vi "KeyToVirtualKey.vi"(11 "keyType Recorded":T1=enum."1") -> (2 "Unimplemented":bool, 3 "Virtual Key":T2=164)   [LabVIEW 2026]
uses:
  replay/KeyboardReplayKey.ctl
  UserEventRecorder/KeyType.ctl
panel:
  in  "\"":bool
  in  ",":bool
  in  ".":bool
  in  "/":bool
  in  "]":bool
  in  "\\":bool
  in  "-":bool
  in  "=":bool
  in  "[":bool
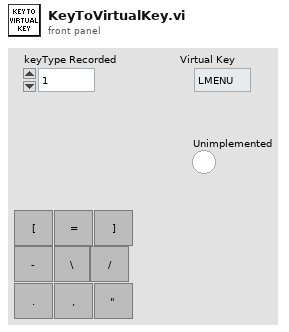
[diagram p1: front panel]
types:
  T1 = typedef "KeyType.ctl" = enum16{"0", "1", "2", "3", "4", "5", "6", "7", "8", "9", "A", "B", "C", "D", "E", "F", "G", "H", "I", "J", "K", "L", "M", "N", "O", "P", "Q", "R", "S", "T", "U", "V", "W", "X", "Y", "Z", "F1", "F2", "F3", "F4", "F5", "F6", "F7", "F8", "F9", "F10", "F11", "F12", "F13", "F14", "F15", "ADD", "BACK", "BACKSLASH", "CAPITAL", "COMMA", "DECIMAL", "DELETE", "DIVIDE", "DOWN", "END", "EQUALS", "ESCAPE", "GRAVE (`)", "HOME", "INSERT", "LBRACKET", "LCONTROL", "LEFT", "L ALT", "LSHIFT", "LWIN", "MINUS", "MULTIPLY", "NEXT", "NUMLOCK", "NUMPAD_0", "NUMPAD_1", "NUMPAD_2", "NUMPAD_3", "NUMPAD_4", "NUMPAD_5", "NUMPAD_6", "NUMPAD_7", "NUMPAD_8", "NUMPAD_9", "PAUSE", "PERIOD", "PRIOR (PG UP)", "RBRACKET", "RCONTROL", "RETURN", "RIGHT", "R ALT", "RSHIFT", "RWIN", "SCROLL", "SEMICOLON", "SLASH", "SPACE", "SUBTRACT", "TAB", "UP", "ENTER (num pad)", "' (quote)"}
  T2 = typedef "KeyboardReplayKey.ctl" = u8
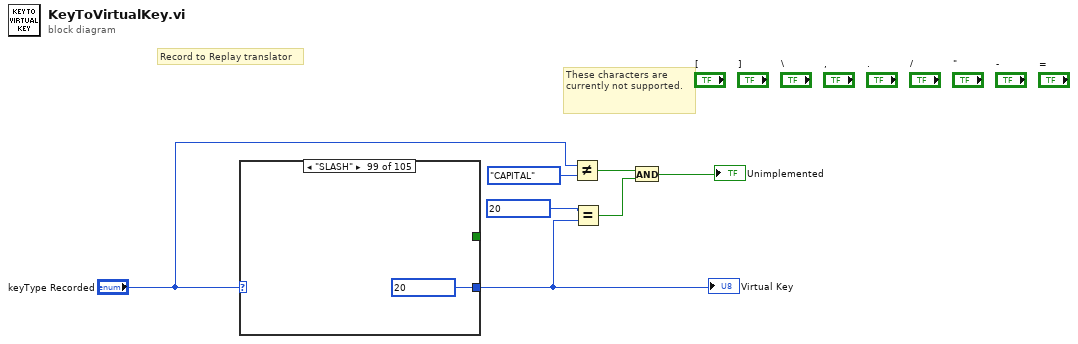
[diagram p0: block diagram]
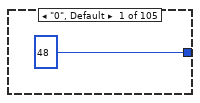
[diagram p2: hidden frame]
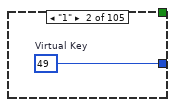
[diagram p3: hidden frame]
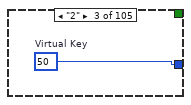
[diagram p4: hidden frame]
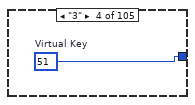
[diagram p5: hidden frame]
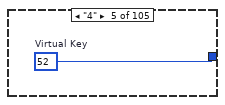
[diagram p6: hidden frame]
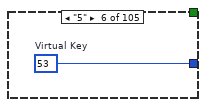
[diagram p7: hidden frame]
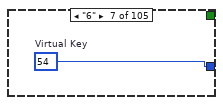
[diagram p8: hidden frame]
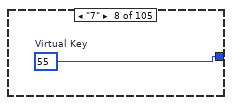
[diagram p9: hidden frame]
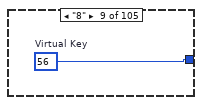
[diagram p10: hidden frame]
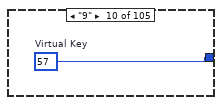
[diagram p11: hidden frame]
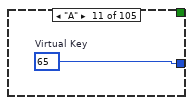
[diagram p12: hidden frame]
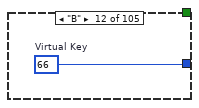
[diagram p13: hidden frame]
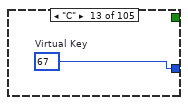
[diagram p14: hidden frame]
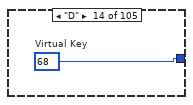
[diagram p15: hidden frame]
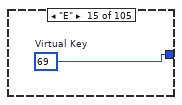
[diagram p16: hidden frame]
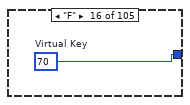
[diagram p17: hidden frame]
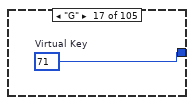
[diagram p18: hidden frame]
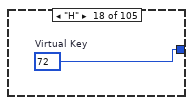
[diagram p19: hidden frame]
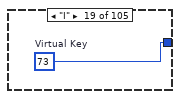
[diagram p20: hidden frame]
diagram:
  # "These characters are\ncurrently not supported."
  # "Record to Replay translator"
  n1 = case shown="\"SLASH\"" "keyType Recorded" {
    tunnel: [T2 48 ("Virtual Key") w9 w10 w11 w12 w13 w14 w15 w16 w17 w18 w19 w20 w21 w22 w23 w24 w25 w26 w27 w28 w29 w30 w31 w32 w33 w34 w35 w36 w37 w38 w39 w40 w41 w42 w43 w44 w45 w46 w47 w48 w49 w50 w51 w52 w53 w54 w55 w56 w57 w58 w59 w60 T2 20 ("Virtual Key") w63 T2 20 ("Virtual Key") w65 w66 w67 w68 w69 T2 20 ("Virtual Key") w71 T2 20 ("Virtual Key") w73 w74 T2 20 ("Virtual Key") w76 w77 w78 T2 160 ("Virtual Key") T2 91 ("Virtual Key") T2 109 ("Virtual Key") T2 106 ("Virtual Key") T2 34 ("Virtual Key") T2 144 ("Virtual Key") T2 96 ("Virtual Key") T2 97 ("Virtual Key") T2 98 ("Virtual Key") T2 99 ("Virtual Key") T2 100 ("Virtual Key") T2 101 ("Virtual Key") T2 102 ("Virtual Key") T2 103 ("Virtual Key") T2 104 ("Virtual Key") T2 105 ("Virtual Key") T2 19 ("Virtual Key") T2 20 ("Virtual Key") T2 33 ("Virtual Key") T2 20 ("Virtual Key") T2 163 ("Virtual Key") T2 43 ("Virtual Key") T2 39 ("Virtual Key") T2 165 ("Virtual Key") T2 161 ("Virtual Key") T2 92 ("Virtual Key") T2 145 ("Virtual Key") T2 164 ("Virtual Key") T2 20 ("Virtual Key") T2 32 ("Virtual Key") T2 109 ("Virtual Key") T2 9 ("Virtual Key") T2 38 ("Virtual Key") T2 20 ("Virtual Key") T2 20 ("Virtual Key")] -> w5
    tunnel: [_ _ _ _ _ _ _ _ _ _ _ _ _ _ _ _ _ _ _ _ _ _ _ _ _ _ _ _ _ _ _ _ _ _ _ _ _ _ _ _ _ _ _ _ _ _ _ _ _ _ _ _ _ w62 _ _ _ _ _ _ _ _ _ _ _ _ _ _ _ _ _ _ _ _ _ _ _ _ _ _ _ _ _ _ _ _ _ _ _ _ _ _ _ _ _ _ _ _ _ _ _ _ _ _ _] -> _
    frame "0", Default {
    }
    frame "1" {
      w9 = T2 49  # Virtual Key
    }
    frame "2" {
      w10 = T2 50  # Virtual Key
    }
    frame "3" {
      w11 = T2 51  # Virtual Key
    }
    frame "4" {
      w12 = T2 52  # Virtual Key
    }
    frame "5" {
      w13 = T2 53  # Virtual Key
    }
    frame "6" {
      w14 = T2 54  # Virtual Key
    }
    frame "7" {
      w15 = T2 55  # Virtual Key
    }
    frame "8" {
      w16 = T2 56  # Virtual Key
    }
    frame "9" {
      w17 = T2 57  # Virtual Key
    }
    frame "A" {
      w18 = T2 65  # Virtual Key
    }
    frame "B" {
      w19 = T2 66  # Virtual Key
    }
    frame "C" {
      w20 = T2 67  # Virtual Key
    }
    frame "D" {
      w21 = T2 68  # Virtual Key
    }
    frame "E" {
      w22 = T2 69  # Virtual Key
    }
    frame "F" {
      w23 = T2 70  # Virtual Key
    }
    frame "G" {
      w24 = T2 71  # Virtual Key
    }
    frame "H" {
      w25 = T2 72  # Virtual Key
    }
    frame "I" {
      w26 = T2 73  # Virtual Key
    }
    frame "J" {
      w27 = T2 74  # Virtual Key
    }
    frame "K" {
      w28 = T2 75  # Virtual Key
    }
    frame "L" {
      w29 = T2 76  # Virtual Key
    }
    frame "M" {
      w30 = T2 77  # Virtual Key
    }
    frame "N" {
      w31 = T2 78  # Virtual Key
    }
    frame "O" {
      w32 = T2 79  # Virtual Key
    }
    frame "P" {
      w33 = T2 80  # Virtual Key
    }
    frame "Q" {
      w34 = T2 81  # Virtual Key
    }
    frame "R" {
      w35 = T2 82  # Virtual Key
    }
    frame "S" {
      w36 = T2 83  # Virtual Key
    }
    frame "T" {
      w37 = T2 84  # Virtual Key
    }
    frame "U" {
      w38 = T2 85  # Virtual Key
    }
    frame "V" {
      w39 = T2 86  # Virtual Key
    }
    frame "W" {
      w40 = T2 87  # Virtual Key
    }
    frame "X" {
      w41 = T2 88  # Virtual Key
    }
    frame "Y" {
      w42 = T2 89  # Virtual Key
    }
    frame "Z" {
      w43 = T2 90  # Virtual Key
    }
    frame "F1" {
      w44 = T2 112  # Virtual Key
    }
    frame "F2" {
      w45 = T2 113  # Virtual Key
    }
    frame "F3" {
      w46 = T2 114  # Virtual Key
    }
    frame "F4" {
      w47 = T2 115  # Virtual Key
    }
    frame "F5" {
      w48 = T2 116  # Virtual Key
    }
    frame "F6" {
      w49 = T2 117  # Virtual Key
    }
    frame "F7" {
      w50 = T2 118  # Virtual Key
    }
    frame "F8" {
      w51 = T2 119  # Virtual Key
    }
    frame "F9" {
      w52 = T2 120  # Virtual Key
    }
    frame "F10" {
      w53 = T2 121  # Virtual Key
    }
    frame "F11" {
      w54 = T2 122  # Virtual Key
    }
    frame "F12" {
      w55 = T2 123  # Virtual Key
    }
    frame "F13" {
      w56 = T2 124  # Virtual Key
    }
    frame "F14" {
      w57 = T2 125  # Virtual Key
    }
    frame "F15" {
      w58 = T2 126  # Virtual Key
    }
    frame "ADD" {
      w59 = T2 107  # Virtual Key
    }
    frame "BACK" {
      w60 = T2 8  # Virtual Key
    }
    frame "BACKSLASH" {
      w62 = TRUE  # Reset
    }
    frame "CAPITAL" {
      w63 = T2 20  # Virtual Key
    }
    frame "COMMA" {
    }
    frame "DECIMAL" {
      w65 = T2 110  # Virtual Key
    }
    frame "DELETE" {
      w66 = T2 46  # Virtual Key
    }
    frame "DIVIDE" {
      w67 = T2 111  # Virtual Key
    }
    frame "DOWN" {
      w68 = T2 40  # Virtual Key
    }
    frame "END" {
      w69 = T2 35  # Virtual Key
    }
    frame "EQUALS" {
    }
    frame "ESCAPE" {
      w71 = T2 27  # Virtual Key
    }
    frame "GRAVE (`)" {
    }
    frame "HOME" {
      w73 = T2 36  # Virtual Key
    }
    frame "INSERT" {
      w74 = T2 45  # Virtual Key
    }
    frame "LBRACKET" {
    }
    frame "LCONTROL" {
      w76 = T2 162  # Virtual Key
    }
    frame "LEFT" {
      w77 = T2 37  # Virtual Key
    }
    frame "L ALT" {
      w78 = T2 164  # Virtual Key
    }
    frame "LSHIFT" {
    }
    frame "LWIN" {
    }
    frame "MINUS" {
    }
    frame "MULTIPLY" {
    }
    frame "NEXT" {
    }
    frame "NUMLOCK" {
    }
    frame "NUMPAD_0" {
    }
    frame "NUMPAD_1" {
    }
    frame "NUMPAD_2" {
    }
    frame "NUMPAD_3" {
    }
    frame "NUMPAD_4" {
    }
    frame "NUMPAD_5" {
    }
    frame "NUMPAD_6" {
    }
    frame "NUMPAD_7" {
    }
    frame "NUMPAD_8" {
    }
    frame "NUMPAD_9" {
    }
    frame "PAUSE" {
    }
    frame "PERIOD" {
    }
    frame "PRIOR (PG UP)" {
    }
    frame "RBRACKET" {
    }
    frame "RCONTROL" {
    }
    frame "RETURN" {
    }
    frame "RIGHT" {
    }
    frame "R ALT" {
    }
    frame "RSHIFT" {
    }
    frame "RWIN" {
    }
    frame "SCROLL" {
    }
    frame "SEMICOLON" {
    }
    frame "SLASH" {
    }
    frame "SPACE" {
    }
    frame "SUBTRACT" {
    }
    frame "TAB" {
    }
    frame "UP" {
    }
    frame "ENTER (num pad)" {
    }
    frame "' (quote)" {
    }
  }
  "Virtual Key" <- w5
  n2 = Not Equal?(x="keyType Recorded", y=KeyType."CAPITAL") -> (x != y?=w3:bool)
  n3 = Equal?(x=T2 20 ("Virtual Key"), y=w5) -> (x = y?=w2:bool)
  n4 = And(x=w3, y=w2) -> (x .and. y?=→"Unimplemented":bool)
